vi "RemoteVI List Top Windows.vi"() -> (4 "windows":T1(array[cluster]))   [LabVIEW 2020, in "RemoteVI.lvlib"]
doc: "Every visible top-level window of the desktop, for RemoteVI Server's list (RemoteVI Window Rows.vi filters and groups them): walks the Z order with user32 FindWindowExW.vi (no callback, at most 4000 windows); for each VISIBLE window its caption (RemoteVI Target Name.vi), class (user32 GetClassNameW.vi), process (user32 GetWindowThreadProcessId.vi) and that process's program path (RemoteVI Process Path.vi), whether it has an owner (user32 GetWindow.vi GW_OWNER), its extended style (GWL_EXSTYLE) and size (user32 GetWindowRect.vi). Win32 only, so it also lists the windows of other programs and of other LabVIEWs."
uses:
  RemoteVI.lvlib
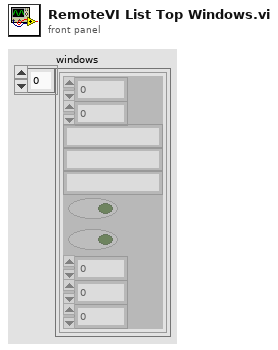
[diagram p1: front panel]
types:
  T1 = cluster{"hWnd":u64, "pid":u32, "path":string, "class":string, "title":string, "visible":bool, "owned":bool, "ex style":u32, "w":i32, "h":i32}[]
  T2 = cluster{"hWnd":u64, "pid":u32, "path":string, "class":string, "title":string, "visible":bool, "owned":bool, "ex style":u32, "w":i32, "h":i32}
  T3 = cluster{"left":i32, "top":i32, "right":i32, "bottom":i32}
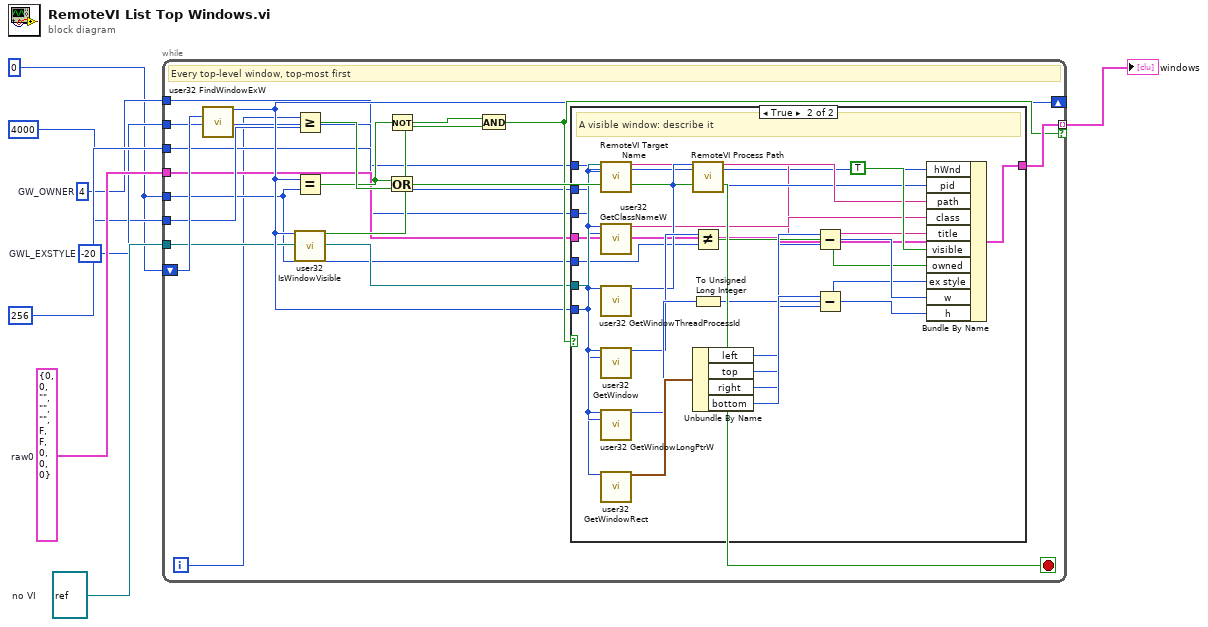
[diagram p0: block diagram]
diagram:
  w7 = refnum<vi> refnum  # no VI
  w6 = T2 {"hWnd"=0, "pid"=0, "path"="", "class"="", "title"="", "visible"=FALSE, "owned"=FALSE, "ex style"=0, "w"=0, "h"=0}  # raw0
  w4 = -20  # GWL_EXSTYLE
  w3 = u32 4  # GW_OWNER
  w1 = u64 0
  n1 = while {
    tunnel: w3 -> [w10]
    tunnel: w4 -> [w11]
    tunnel: 256 -> [w12]
    tunnel: w6 -> [w13]
    tunnel: w1 -> [w14]
    tunnel: 4000 -> [w15]
    tunnel: w7 -> [w16]
    shift-right: [w18] -> _
    shift-left: w1 -> [w17]
    tunnel: [w23] -> w8 mode=indexing if=w22
    i -> [w9]
    stop <- w25 stop-if-true
    # "Every top-level window, top-most first"
    n2 = call "user32 FindWindowExW.vi"("hWndChildAfter"=w17) -> ("hWnd"=w18:u64)  [unwired: 13 in, 1 out]
    n3 = Greater Or Equal?(x=w9, y=w15) -> (x >= y?=w24:bool)
    n4 = Equal?(x=w18, y=w14) -> (x = y?=w19:bool)
    n5 = call "user32 IsWindowVisible.vi"("hWnd"=w18) -> ("visible?"=w20:bool)  [unwired: 13 in, 1 out]
    n6 = Not(x=w19) -> (.not. x?=w21:bool)
    n7 = Or(x=w19, y=w24) -> (x .or. y?=w25:bool)
    n8 = And(x=w21, y=w20) -> (x .and. y?=w22:bool)
    n9 = case shown="True" w22 {
      tunnel: w10 -> [_ w28]
      tunnel: w11 -> [_ w29]
      tunnel: w12 -> [_ w30]
      tunnel: w13 -> [w26 w31]
      tunnel: w14 -> [_ w32]
      tunnel: w16 -> [_ w33]
      tunnel: w18 -> [_ w27]
      tunnel: [w26 w50] -> w23
      frame False {
      }
      frame True {
        # "A visible window: describe it"
        n10 = call "RemoteVI Target Name.vi"("VI"=w33, "window"=w27) -> ("name"=w34:string)  [unwired: 12 in, 1 out]
        n11 = call "user32 GetClassNameW.vi"("hWnd"=w27, "nMaxCount"=w30) -> ("class name"=w35:string)  [unwired: 11 in, 2 out]
        n12 = call "user32 GetWindowThreadProcessId.vi"("hWnd"=w27) -> ("process ID"=w36:u32)  [unwired: 12 in, 2 out]
        n13 = call "user32 GetWindow.vi"("hWnd"=w27, "uCmd"=w28) -> ("window"=w38:u64)  [unwired: 12 in, 1 out]
        n14 = call "user32 GetWindowLongPtrW.vi"("hWnd"=w27, "nIndex"=w29) -> ("return value"=w40:i64)  [unwired: 12 in, 1 out]
        n15 = call "user32 GetWindowRect.vi"("hWnd"=w27) -> ("RECT"=w42:T3)  [unwired: 12 in, 2 out]
        n16 = call "RemoteVI Process Path.vi"("process ID"=w36) -> ("path"=w37:string)  [unwired: 14 in]
        n17 = Not Equal?(x=w38, y=w32) -> (x != y?=w39:bool)
        n18 = To Unsigned Long Integer(number=w40) -> (unsigned 32bit integer=w41:u32)
        n19 = Unbundle By Name(w42) -> ("left"=w43:i32, "top"=w44:i32, "right"=w45:i32, "bottom"=w46:i32)
        n20 = Subtract(x=w45, y=w43) -> (x-y=w47:i32)
        n21 = Subtract(x=w46, y=w44) -> (x-y=w48:i32)
        n22 = Bundle By Name(cluster=w31, "hWnd"=w27, "pid"=w36, "path"=w37, "class"=w35, "title"=w34, "visible"=TRUE, "owned"=w39, "ex style"=w41, "w"=w47, "h"=w48) -> (w50:T2)
      }
    }
  }
  "windows" <- w8
